vi "[ce] Levenberg Marquardt.vi"(0 "X":dbl[](array[numeric]) format="%.2f", 1 "Standard Deviation":dbl[](array[numeric]) format="%.2f", 2 "VC Handle":T1=-1, 5 "Y":dbl[](array[numeric]) format="%.2f", 7 "Initial Guess Coefficients":dbl[](array[numeric]) format="%.2f", 9 "max iteration":i32=200, 11 "error in":errorcluster, 12 "model description":T2) -> (3 "Covariance":dbl[][](array[numeric]) format="%.2f", 4 "Best Fit Coefficients":dbl[](array[numeric]) format="%.2f", 6 "Best Fit":dbl[](array[numeric]) format="%.2f", 8 "mse":dbl format="%.4e", 10 "ticks":u32, 14 "iterations":i32, 15 "error out":errorcluster)   [LabVIEW 2021]
doc: "This VI uses the Levenberg-Marquardt algorithm to determine the least squares set of coefficients that best fit the set of input data points (<b>X</b>, <b>Y</b>) as expressed by a nonlinear function <b>y = f(x, a)</b> where <b>a</b> is the set of coefficients.\n\n::: CalcExpress Toolkit :::\nCopyright (c) 2000-2026 Konstantin Shifershteyn. All rights reserved."
uses:
  [ce] LM Fit - model description.ctl
  cetypes.llb/VarMan Variable Context Handle.ctl
  <vilib>/Analysis/baseanly.llb/Real Inverse Matrix.vi
  <vilib>/Analysis/NI_AALBase.lvlib
panel:
  # "Nonlinear  Levenberg Marquardt  Fit\n[CalcExpress version]"
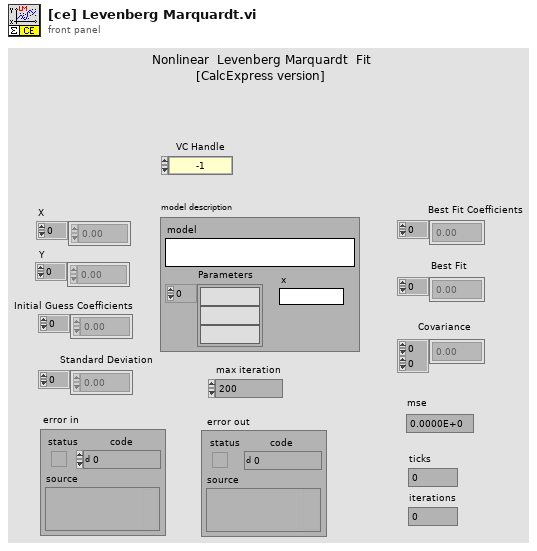
[diagram p1: front panel]
types:
  T1 = typedef "VarMan Variable Context Handle.ctl" = i32
  T2 = typedef "[ce] LM Fit - model description.ctl" = cluster{"model":string, "Parameters":string[], "x":string}
  T3 = typedef "NI_Matrix.lvlib/RealMatrix.ctl" = dbl[][]
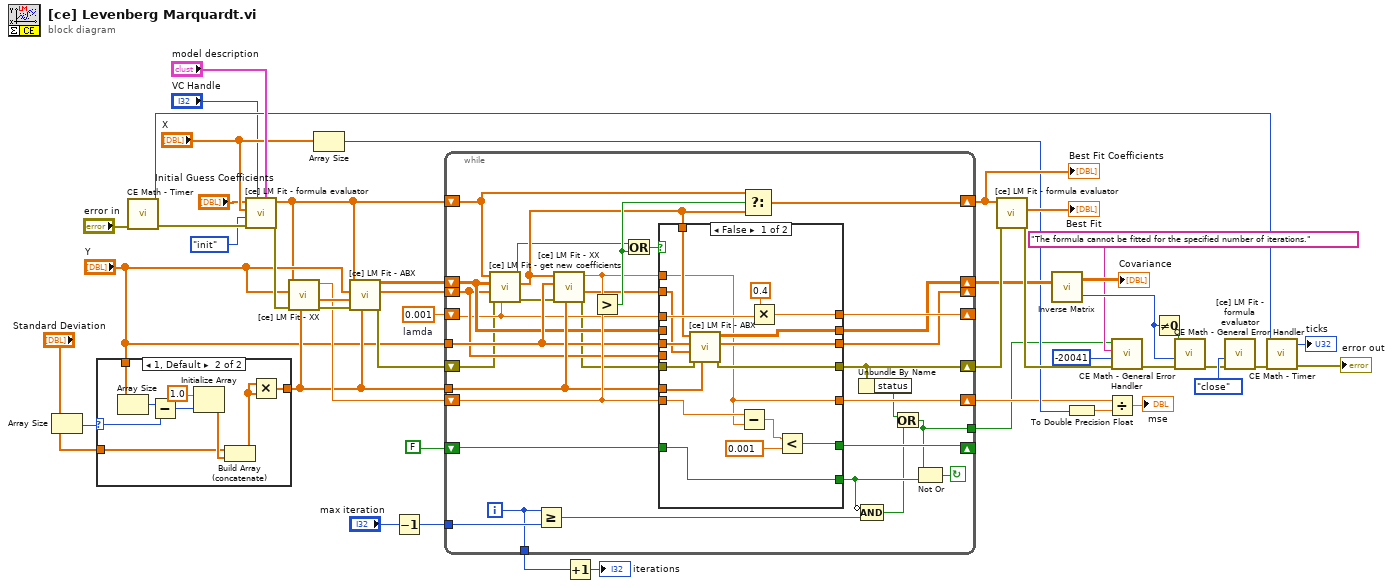
[diagram p0: block diagram]
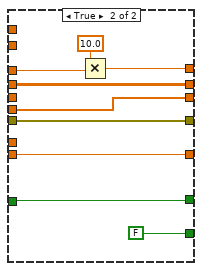
[diagram p3: hidden frame]
diagram:
  w46 = 0.001  # lamda
  n1 = Array Size(array="Standard Deviation") -> (size(s)=w3:i32)
  n2 = case shown="1, Default" w3 {
    selector: w3 -> [_ w49]
    tunnel: "Standard Deviation" -> [w48 w53]
    tunnel: [w48 w51] -> w35
    tunnel: "Y" -> [_ w50]
    frame 0 {
    }
    frame 1, Default {
      n3 = Array Size(array=w50) -> (size(s)=w56:i32)
      n4 = Subtract(x=w56, y=w49) -> (x-y=w55:i32)
      n5 = Initialize Array(1.0, w55) -> (w54:dbl[])
      n6 = Build Array (concatenate)(w53, w54) -> (w52:dbl[])
      n7 = Multiply(x=w52, y=w52) -> (x*y=w51:dbl[])
    }
  }
  n8 = call "CE Math - Timer.vi"("error in (no error)"="error in") -> ("error out"=w29:errorcluster, "ticks out"=w24:u32)  [unwired: 7 in]
  n9 = call "[ce] LM Fit - formula evaluator.vi"("formula params"="model description", "VC Handle"="VC Handle", "error in"=w29, "action"=enum16{"init", "close", "calculate"}."init", "X (for init only)"="X", "coef values"="Initial Guess Coefficients") -> ("error out"=w38:errorcluster, "coef values out"=w31:dbl[])  [unwired: 3 in, 1 out]
  n10 = call "[ce] LM Fit - XX.vi"("Standard Deviation ^2"=w35, "error in"=w38, "Y"="Y", "coefficient values"=w31) -> ("error out"=w39:errorcluster, "calc formula result"=w37:dbl[], "chiSqr"=w36:dbl)  [unwired: 3 in]
  n11 = Array Size(array="X") -> (size(s)=w9:i32)
  n12 = call "[ce] LM Fit - ABX.vi"("Standard Deviation ^2"=w35, "error in"=w39, "data for given coefficients"=w37, "Y"="Y", "coefficient values"=w31) -> ("error out"=w41:errorcluster, "Beta"=w45:dbl[], "Alpha"=w47:dbl[][])  [unwired: 2 in]
  n13 = Decrement(x="max iteration") -> (x-1=w33:i32)
  n14 = while {
    tunnel: [w62] -> w4
    shift-left: w41 -> [w69]
    shift-right: [w65] -> w18
    tunnel: "Y" -> [w82]
    tunnel: w33 -> [w66]
    tunnel: w35 -> [w83]
    shift-left: FALSE -> [w85]
    shift-right: [w84] -> _
    shift-left: w36 -> [w86]
    shift-right: [w87] -> w8
    shift-left: w45 -> [w80]
    shift-right: [w88] -> _
    shift-left: w47 -> [w81]
    shift-right: [w77] -> w12
    shift-left: w31 -> [w72]
    shift-right: [w75] -> w20
    shift-left: w46 -> [w79]
    shift-right: [w89] -> _
    tunnel: [w58] -> w1
    i -> [w58]
    stop <- w63 continue-if-true
    n15 = call "[ce] LM Fit - get new coefficients.vi"("lamda"=w79, "error in"=w69, "Beta"=w80, "Alpha"=w81, "Coefficients"=w72) -> ("error out"=w68:errorcluster, "New Coefficients"=w73:dbl[], "err flag"=w67:bool)  [unwired: 4 in]
    n16 = Greater Or Equal?(x=w58, y=w66) -> (x >= y?=w60:bool)
    n17 = call "[ce] LM Fit - XX.vi"("Standard Deviation ^2"=w83, "error in"=w68, "Y"=w82, "coefficient values"=w73) -> ("error out"=w78:errorcluster, "calc formula result"=w70:dbl[], "chiSqr"=w71:dbl)  [unwired: 3 in]
    n18 = Greater?(x=w71, y=w86) -> (0:w74:bool)
    n19 = Or(x=w67, y=w74) -> (x .or. y?=w76:bool)
    n20 = case shown="False" w76 {
      tunnel: w79 -> [w105 w114]
      tunnel: [w104 w113] -> w89
      tunnel: [w97 w112] -> w77
      tunnel: w81 -> [_ w112]
      tunnel: [w98 w108] -> w88
      tunnel: [w95 w111] -> w87
      tunnel: w86 -> [w103 w111]
      tunnel: w85 -> [w93 w110]
      tunnel: [w91 w110] -> w84
      tunnel: [w93 FALSE] -> w61
      tunnel: w80 -> [_ w108]
      tunnel: w83 -> [w99 _]
      tunnel: w82 -> [w100 _]
      tunnel: w78 -> [w102 w107]
      tunnel: [w101 w107] -> w65
      tunnel: w73 -> [w96 _]
      tunnel: w71 -> [w95 _]
      tunnel: w70 -> [w94 _]
      frame False {
        n21 = call "[ce] LM Fit - ABX.vi"("Standard Deviation ^2"=w99, "error in"=w102, "data for given coefficients"=w94, "Y"=w100, "coefficient values"=w96) -> ("error out"=w101:errorcluster, "Beta"=w98:dbl[], "Alpha"=w97:dbl[][])  [unwired: 2 in]
        n22 = Subtract(x=w103, y=w95) -> (x-y=w92:dbl)
        n23 = Multiply(x=0.4, y=w105) -> (x*y=w104:dbl)
        n24 = Less?(x=w92, y=0.001) -> (x < y?=w91:bool)
      }
      frame True {
        n25 = Multiply(x=10.0, y=w114) -> (x*y=w113:dbl)
      }
    }
    n26 = Select(t=w72, s=w74, f=w73) -> (s? t:f=w75:dbl[])
    n27 = Unbundle By Name(w65) -> ("status"=w64:bool)
    n28 = Compound Arithmetic op=AND(invert w61, w60) -> (w59:bool)
    n29 = Or(x=w64, y=w59) -> (x .or. y?=w62:bool)
    n30 = Not Or(1:w61, 2:w62) -> (0:w63:bool)
  }
  "Best Fit Coefficients" <- w20
  n31 = Increment(x=w1) -> (x+1=→"iterations":i32)
  n32 = call "[ce] LM Fit - formula evaluator.vi"("error in"=w18, "coef values"=w20) -> ("error out"=w17:errorcluster, "calc result"=→"Best Fit":dbl[])  [unwired: 7 in, 1 out]
  n33 = call-poly <vilib>:"Inverse Matrix.vi"("Input Matrix"=w12) -> ("error"=w15:i32, "Inverse Matrix"=→"Covariance":T3)  [unwired: 1 in]
  n34 = To Double Precision Float(number=w9) -> (double precision float=w10:dbl)
  n35 = Divide(x=w8, y=w10) -> (x/y=→"mse":dbl)
  n36 = call "CE Math - General Error Handler.vi"("error before"=w17, "error code"=-20041 ("error code (no error:0)"), "message"="The formula cannot be fitted for the specified number of iterations.", "error? (T)"=w4) -> ("error out"=w13:errorcluster)  [unwired: 4 in, 1 out]
  n37 = Not Equal To 0?(x=w15) -> (x != 0?=w16:bool)
  n38 = call "CE Math - General Error Handler.vi"("error before"=w13, "error code"=w15, "error? (T)"=w16) -> ("error out"=w14:errorcluster)  [unwired: 5 in, 1 out]
  n39 = call "[ce] LM Fit - formula evaluator.vi"("error in"=w14, "action"=enum16{"init", "close", "calculate"}."close") -> ("error out"=w27:errorcluster)  [unwired: 7 in, 2 out]
  n40 = call "CE Math - Timer.vi"("error in (no error)"=w27, "ticks in"=w24) -> ("error out"=→"error out":errorcluster, "ticks out"=→"ticks":u32)  [unwired: 6 in]
